vi "VIH HelpGen - Write HTML File - Poly VI - VI Description.vi"(4 "Templates":T3, 6 "Description Params":cluster{"DscrMode":T5, "Description":string}, 7 "Save params":T1, 8 "error in":errorcluster, 9 "Project Tree":T4, 10 "HTML in":string, 11 "VI Reference":refnum<vi>) -> (0 "error out":errorcluster, 1 "VI Name":string, 2 "HTML out":string, 3 "dup VI Reference":refnum<vi>)   [LabVIEW 2014]
doc: "::: VI Helpeks :::\nCopyright (c) 2000-2026 Konstantin Shifershteyn. All rights reserved."
uses:
  VIH HelpGen Typedef - Enum - Description Mode.ctl
  _VIH Project Manager.llb/VIH Project Tree Typedef - Tree Refnum.ctl
  VIH HelpGen Typedef - Table Templates Cluster - VI Help.ctl
panel:
  # "VI Helpeks\nCopyright (c) 2012-2026 Konstantin Shifershteyn"
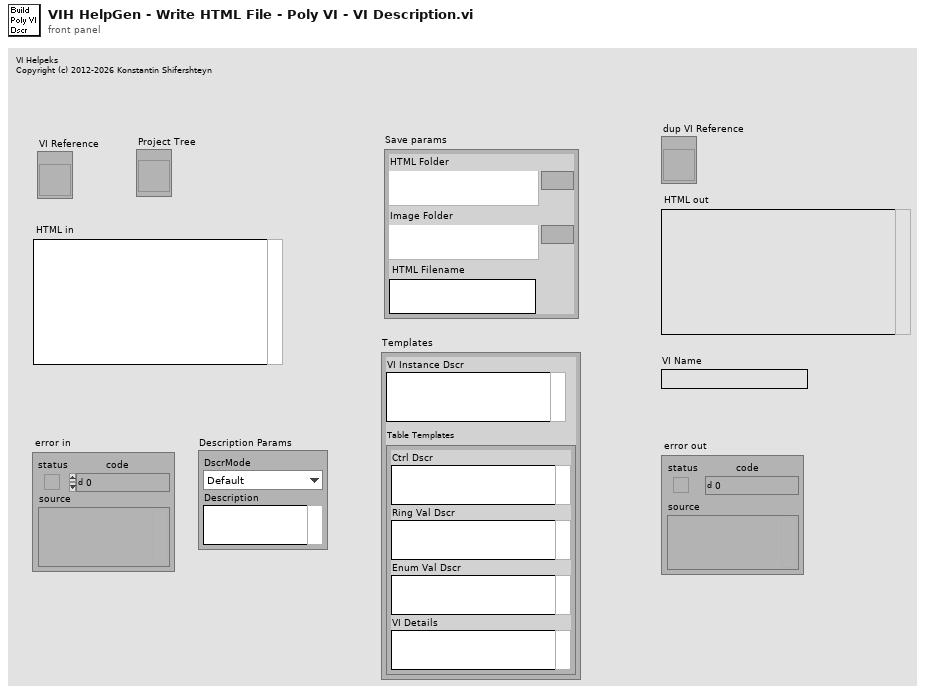
[diagram p1: front panel]
types:
  T1 = cluster{"HTML Folder":path, "Image Folder":path, "HTML Filename":string}
  T2 = typedef "VIH HelpGen Typedef - Table Templates Cluster - VI Help.ctl" = cluster{"Ctrl Dscr":string, "Ring Val Dscr":string, "Enum Val Dscr":string, "VI Details":string}
  T3 = cluster{"VI Instance Dscr":string, "Table Templates":T2}
  T4 = typedef "VIH Project Tree Typedef - Tree Refnum.ctl" = refnum<vi>
  T5 = typedef "VIH HelpGen Typedef - Enum - Description Mode.ctl" = enum16{"Default", "Description", "Description1", "Description2", "Custom", "None"}
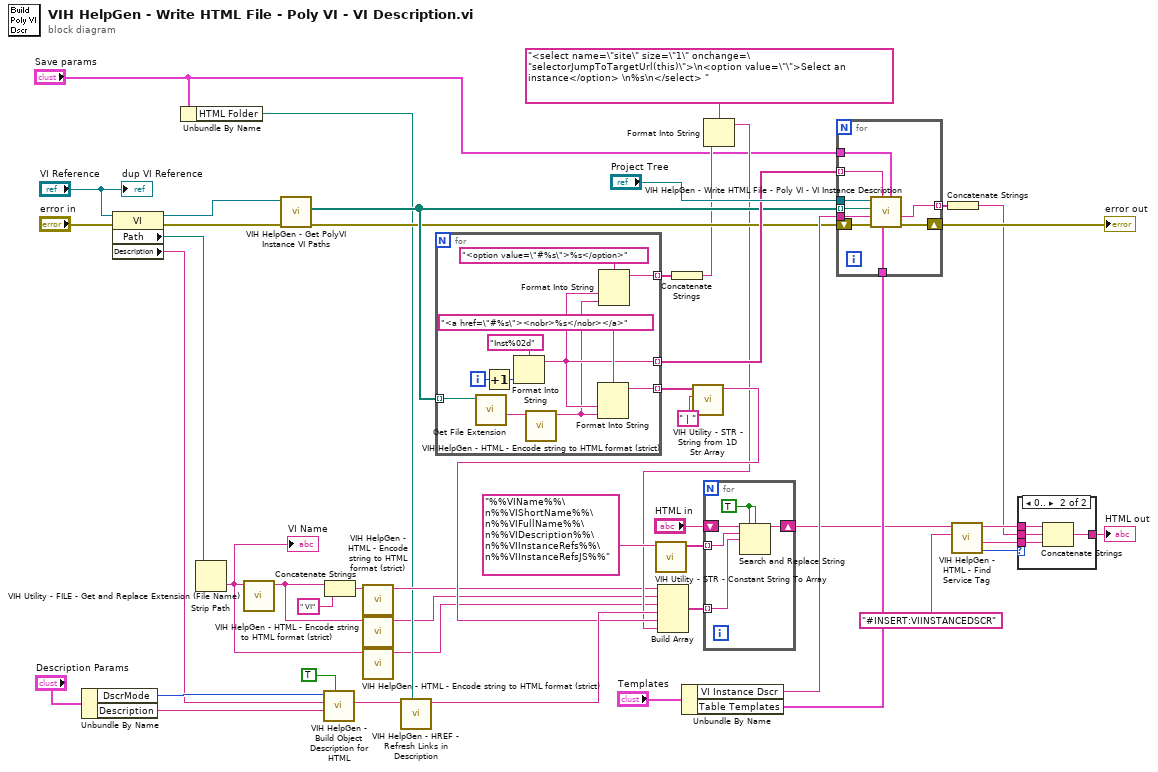
[diagram p0: block diagram]
diagram:
  n1 = Unbundle By Name("Description Params") -> ("DscrMode"=w42:T5, "Description"=w40:string)
  n2 = property class="VI"(reference="VI Reference", error in="error in") -> (reference out=w16:refnum<vi>, error out=w15:errorcluster, "Path"=w36:path, "Description"=w41:string)
  n3 = Unbundle By Name("Save params") -> ("HTML Folder"=w6:path)
  n4 = Strip Path(path=w36) -> (name=w5:string)  [unwired: 1 out]
  "VI Name" <- w5
  n5 = call "VIH Utility - FILE - Get and Replace Extension (File Name).vi"("File name"=w5) -> ("File name out"=w2:string)  [unwired: 9 in, 1 out]
  n6 = call "VIH HelpGen - Get PolyVI Instance VI Paths.vi"("error in"=w15, "VI Reference"=w16) -> ("error out"=w13:errorcluster, "Instance VI Paths"=w14:path[])  [unwired: 7 in, 1 out]
  n7 = call "VIH HelpGen - Build Object Description for HTML.vi"("Ena \"No Description\" message (F)"=TRUE ("Ena \"No Description\" message (F)"), "Custom Description"=w40, "Default Description"=w41, "DscrMode"=w42) -> ("Description HTML out"=w38:string)  [unwired: 6 in, 1 out]
  n8 = Concatenate Strings(w2, " VI") -> (w3:string)
  n9 = call "VIH HelpGen - HTML - Encode string to HTML format (strict).vi"("string"=w3) -> ("HTML string"=w8:string)  [unwired: 10 in]
  n10 = call "VIH HelpGen - HTML - Encode string to HTML format (strict).vi"("string"=w2) -> ("HTML string"=w1:string)  [unwired: 10 in]
  n11 = call "VIH HelpGen - HTML - Encode string to HTML format (strict).vi"("string"=w5) -> ("HTML string"=w4:string)  [unwired: 10 in]
  n12 = call "VIH HelpGen - HREF - Refresh Links in Description.vi"("HTML Folder"=w6, "Description in"=w38) -> ("Description out"=w37:string)  [unwired: 9 in]
  n13 = for {
    tunnel: w14 -> [w59] mode=indexing
    tunnel: [w52] -> w29 mode=indexing
    tunnel: [w54] -> w28 mode=indexing
    tunnel: [w51] -> w12 mode=indexing
    i -> [w56]
    n14 = call <vilib>:"Get File Extension.vi"("file"=w59) -> ("filename without extension"=w50:string)  [unwired: 7 in, 3 out]
    n15 = Increment(x=w56) -> (x+1=w55:i32)
    n16 = Format Into String(format string="Inst%02d", w55) -> (resulting string=w52:string)  [unwired: 2 in, 1 out]
    n17 = call "VIH HelpGen - HTML - Encode string to HTML format (strict).vi"("string"=w50) -> ("HTML string"=w49:string)  [unwired: 10 in]
    n18 = Format Into String(format string="<a href=\"#%s\"><nobr>%s</nobr></a>", w52, w49) -> (resulting string=w54:string)  [unwired: 2 in, 1 out]
    n19 = Format Into String(format string="<option value=\"#%s\">%s</option>", w52, w49) -> (resulting string=w51:string)  [unwired: 2 in, 1 out]
  }
  n20 = call "VIH Utility - STR - Constant String To Array.vi"("String in"="%%VIName%%\n%%VIShortName%%\n%%VIFullName%%\n%%VIDescription%%\n%%VIInstanceRefs%%\n%%VIInstanceRefsJS%%") -> ("Array out"=w46:string[])  [unwired: 10 in]
  n21 = Concatenate Strings(w12) -> (w11:string)
  n22 = Unbundle By Name("Templates") -> ("VI Instance Dscr"=w30:string, "Table Templates"=w31:T2)
  n23 = call "VIH Utility - STR - String from 1D Str Array.vi"("delimiter ('\\n')"=" | ", "Array in"=w28) -> ("String out"=w27:string)  [unwired: 5 in]
  n24 = Format Into String(format string="<select name=\"site\" size=\"1\" onchange=\"selectorJumpToTargetUrl(this)\">\n<option value=\"\">Select an instance</option> \n%s\n</select> ", w11) -> (resulting string=w9:string)  [unwired: 2 in, 1 out]
  n25 = Build Array(w8, w1, w4, w37, w27, w9) -> (w45:string[])
  n26 = for {
    shift-right: [w63] -> w21
    shift-left: "HTML in" -> [w64]
    tunnel: w46 -> [w61] mode=indexing
    tunnel: w45 -> [w60] mode=indexing
    w62 = TRUE
    n27 = Search and Replace String(replace all?=w62, case sensitive?=w62, input string=w64, search string=w61, replace string=w60) -> (result string=w63:string)  [unwired: 3 in, 3 out]
  }
  n28 = for {
    tunnel: "Project Tree" -> [w73]
    tunnel: w31 -> [w72]
    shift-right: [w71] -> w34
    shift-left: w13 -> [w70]
    tunnel: w14 -> [w69] mode=indexing
    tunnel: "Save params" -> [w68]
    tunnel: [w67] -> w19 mode=indexing
    tunnel: w30 -> [w66]
    tunnel: w29 -> [w65] mode=indexing
    n29 = call "VIH HelpGen - Write HTML File - Poly VI - VI Instance Description.vi"("Save params"=w68, "Table Templates"=w72, "InstanceRef"=w65, "error in"=w70, "HTML in"=w66, "VI Path"=w69, "Project Tree"=w73) -> ("error out"=w71:errorcluster, "HTML out"=w67:string)  [unwired: 2 in, 1 out]
  }
  "error out" <- w34
  n30 = Concatenate Strings(w19) -> (w18:string)
  n31 = call "VIH HelpGen - HTML - Find Service Tag.vi"("Tag name"="#INSERT:VIINSTANCEDSCR", "HTML in"=w21) -> ("Offset out"=w25:i32, "After"=w24:string, "Before"=w23:string)  [unwired: 6 in, 1 out]
  n32 = case shown="0.." w25 {
    tunnel: w23 -> [w74 w78]
    tunnel: w24 -> [_ w77]
    tunnel: [w74 w76] -> w20
    tunnel: w18 -> [_ w75]
    frame ..-1 {
    }
    frame 0.. {
      n33 = Concatenate Strings(w78, w75, w77) -> (w76:string)
    }
  }
  "HTML out" <- w20
  "dup VI Reference" <- "VI Reference"
